vi "SEQU_ChoixGrappe Complete_CN.vi"(3 "indice grappe":u8) -> (1 "Chaîne au format E":string)   [LabVIEW 2022 SP3]
uses:
  TypeDef_Seuil Jauge Pression_CN.ctl
  Voie Analogique_CN.ctl
  Emum Type Jauge de Pression_CN.ctl
  Variables globales/Variable glob Edwards.vi
  Variables globales/Variable glob generale.vi
panel:
  out "Valeur retenue":T1
  out "Seuil Jauge":T3={"Descente en Pression"={"Min Mesure Piezo"=5.0, "Min Mesure Pirani"=0.0002}, "Montée en Pression"={"Max Mesure Pirani"=10.0, "Max Mesure Penning"=0.0004}} {"Montée en Pression"."Max Mesure Penning" format="%.2e"; "Montée en Pression"."Max Mesure Pirani" format="%.2e"; "Descente en Pression"."Min Mesure Pirani" format="%.2e"; "Descente en Pression"."Min Mesure Piezo" format="%.2e"}
  out "Valeurs lues":dbl[](array[numeric])=[1000.0, 1000.0, 4e-10] format="%#_6e"
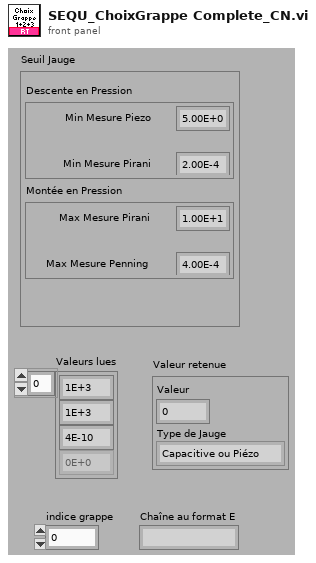
[diagram p1: front panel]
types:
  T1 = typedef "Voie Analogique_CN.ctl" = cluster{"Valeur":dbl, "Type de Jauge":T2}
  T2 = typedef "Emum Type Jauge de Pression_CN.ctl" = enum16{"Capacitive ou Piézo", "Pirani", "Penning"}
  T3 = typedef "TypeDef_Seuil Jauge Pression_CN.ctl" = cluster{"Descente en Pression":cluster{"Min Mesure Piezo":dbl, "Min Mesure Pirani":dbl}, "Montée en Pression":cluster{"Max Mesure Pirani":dbl, "Max Mesure Penning":dbl}}
  T4 = enum16{"Capacitive ou Piézo", "Pirani", "Penning"}
  T5 = enum16{"Capacitive ou Piézo", "Pirani", "Penning", "Bayard Alpert"}
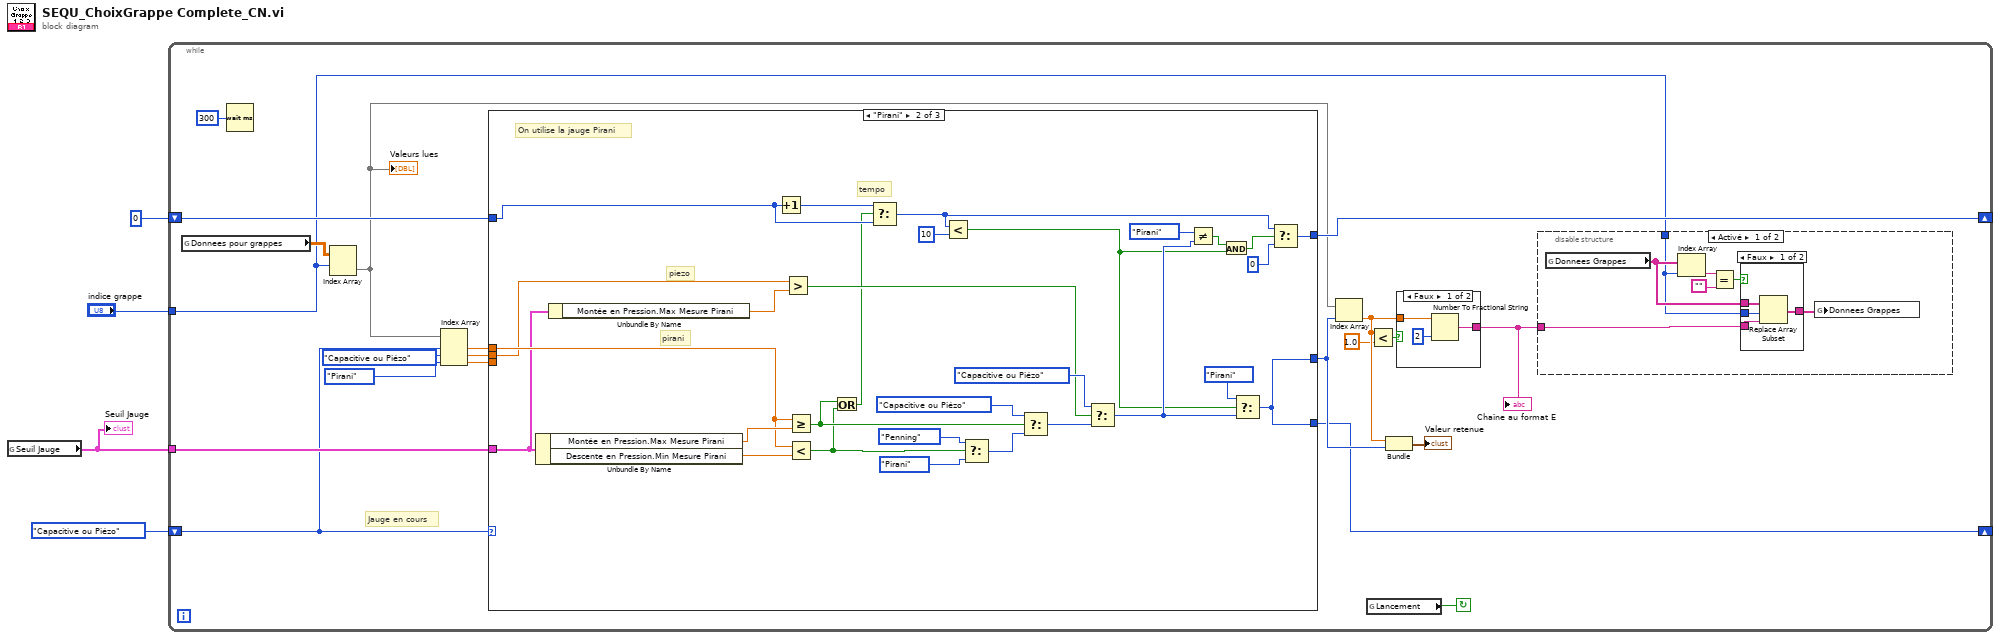
[diagram p0: block diagram]
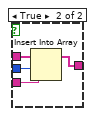
[diagram p2: hidden frame]
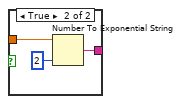
[diagram p4: hidden frame]
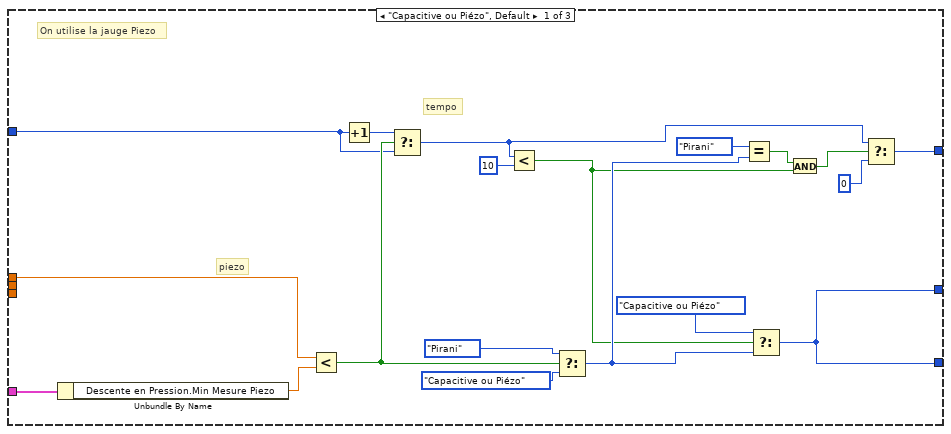
[diagram p5: hidden frame]
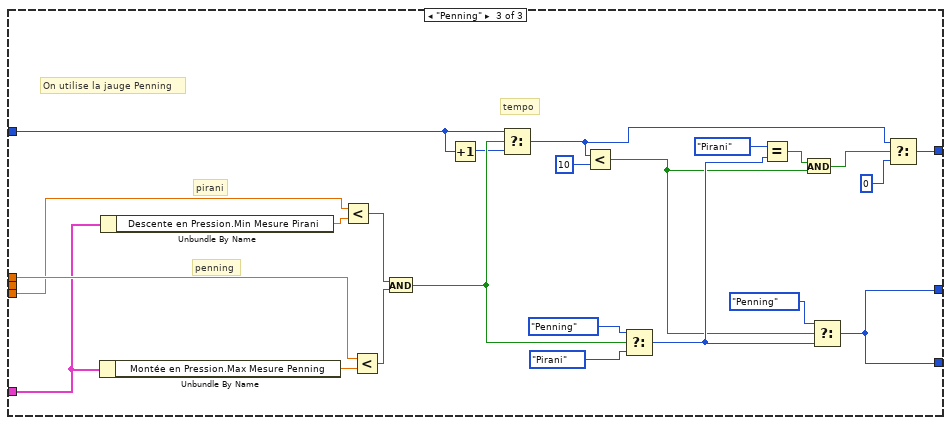
[diagram p6: hidden frame]
diagram:
  n1 = global read "Variable glob Edwards.vi" "Seuil Jauge"() -> (w2:T3)
  "Seuil Jauge" <- w2
  n2 = while {
    tunnel: w2 -> [w25]
    shift-right: [w15] -> _
    shift-left: T4."Capacitive ou Piézo" ("Jauge In") -> [w24]
    shift-right: [w13] -> _
    shift-left: 0 -> [w14]
    tunnel: "indice grappe" -> [w5]
    stop <- w12 continue-if-true
    # "Jauge en cours"
    n3 = global read "Variable glob Edwards.vi" "Donnees pour grappes"() -> (w11:dbl[][])
    n4 = Wait (ms)(milliseconds to wait=u32 300 ("n millisecondes")) -> ()  [unwired: 1 out]
    n5 = Index Array(array=w11, index (row)=w5) -> (element=w10:dbl[])  [unwired: 1 in]
    "Valeurs lues" <- w10
    n6 = Index Array(array=w10, index #1=w24, index #2=T5."Capacitive ou Piézo" ("Jauge In 2"), index #3=T5."Pirani" ("Jauge In 2")) -> (element #1=w23:dbl, element #2=w20:dbl, element #3=w19:dbl)
    n7 = case shown="\"Pirani\"" w24 {
      tunnel: w25 -> [w65 w82 w113]
      tunnel: [w58 w74 w107] -> w16
      tunnel: [w58 w74 w107] -> w15
      tunnel: w23 -> [w61 w88 w114]
      tunnel: w20 -> [_ w86 _]
      tunnel: w19 -> [_ _ w105]
      tunnel: w14 -> [w55 w76 w99]
      tunnel: [w53 w75 w106] -> w13
      frame "Capacitive ou Piézo", Default {
        # "tempo"
        # "piezo"
        # "On utilise la jauge Piezo"
        n8 = Unbundle By Name(w65) -> ("Descente en Pression.Min Mesure Piezo"=w64:dbl)
        n9 = Less?(x=w61, y=w64) -> (x < y?=w57:bool)
        n10 = Increment(x=w55) -> (x+1=w56:i32)
        n11 = Select(t=w56, s=w57, f=w55) -> (s? t:f=w51:i32)
        n12 = Less?(x=w51, y=10) -> (x < y?=w48:bool)
        n13 = Select(t=Emum_Type_Jauge_de_Pression_CN."Pirani" ("Type de Jauge"), s=w57, f=Emum_Type_Jauge_de_Pression_CN."Capacitive ou Piézo" ("Type de Jauge")) -> (s? t:f=w50:T2)
        n14 = Equal?(x=Emum_Type_Jauge_de_Pression_CN."Pirani", y=w50) -> (x = y?=w49:bool)
        n15 = Select(t=Emum_Type_Jauge_de_Pression_CN."Capacitive ou Piézo" ("cas vrai"), s=w48, f=w50) -> (s? t:f=w58:T2)
        n16 = And(x=w49, y=w48) -> (x .and. y?=w47:bool)
        n17 = Select(t=w51, s=w47, f=0 ("cas vrai")) -> (s? t:f=w53:i32)
      }
      frame "Pirani" {
        # "tempo"
        # "piezo"
        # "pirani"
        # "On utilise la jauge Pirani"
        n18 = Unbundle By Name(w82) -> ("Montée en Pression.Max Mesure Pirani"=w94:dbl, "Descente en Pression.Min Mesure Pirani"=w89:dbl)
        n19 = Unbundle By Name(w82) -> ("Montée en Pression.Max Mesure Pirani"=w87:dbl)
        n20 = Increment(x=w76) -> (x+1=w80:i32)
        n21 = Greater?(x=w86, y=w87) -> (0:w73:bool)
        n22 = Greater Or Equal?(x=w88, y=w94) -> (x >= y?=w71:bool)
        n23 = Less?(x=w88, y=w89) -> (x < y?=w70:bool)
        n24 = Or(x=w71, y=w70) -> (x .or. y?=w69:bool)
        n25 = Select(t=w80, s=w69, f=w76) -> (s? t:f=w77:i32)
        n26 = Less?(x=w77, y=10) -> (x < y?=w67:bool)
        n27 = Select(t=Emum_Type_Jauge_de_Pression_CN."Penning" ("Type de Jauge"), s=w70, f=Emum_Type_Jauge_de_Pression_CN."Pirani" ("Type de Jauge")) -> (s? t:f=w92:T2)
        n28 = Select(t=Emum_Type_Jauge_de_Pression_CN."Capacitive ou Piézo" ("Type de Jauge"), s=w71, f=w92) -> (s? t:f=w85:T2)
        n29 = Select(t=Emum_Type_Jauge_de_Pression_CN."Capacitive ou Piézo" ("Type de Jauge"), s=w73, f=w85) -> (s? t:f=w72:T2)
        n30 = Not Equal?(x=Emum_Type_Jauge_de_Pression_CN."Pirani", y=w72) -> (x != y?=w68:bool)
        n31 = And(x=w68, y=w67) -> (x .and. y?=w66:bool)
        n32 = Select(t=Emum_Type_Jauge_de_Pression_CN."Pirani" ("cas vrai"), s=w67, f=w72) -> (s? t:f=w74:T2)
        n33 = Select(t=w77, s=w66, f=0 ("cas vrai")) -> (s? t:f=w75:i32)
      }
      frame "Penning" {
        # "tempo"
        # "pirani"
        # "penning"
        # "On utilise la jauge Penning"
        n34 = Unbundle By Name(w113) -> ("Montée en Pression.Max Mesure Penning"=w115:dbl)
        n35 = Unbundle By Name(w113) -> ("Descente en Pression.Min Mesure Pirani"=w104:dbl)
        n36 = Less?(x=w105, y=w104) -> (x < y?=w103:bool)
        n37 = Less?(x=w114, y=w115) -> (x < y?=w102:bool)
        n38 = And(x=w103, y=w102) -> (x .and. y?=w101:bool)
        n39 = Increment(x=w99) -> (x+1=w100:i32)
        n40 = Select(t=w99, s=w101, f=w100) -> (s? t:f=w108:i32)
        n41 = Less?(x=w108, y=10) -> (x < y?=w96:bool)
        n42 = Select(t=Emum_Type_Jauge_de_Pression_CN."Penning" ("Type de Jauge"), s=w101, f=Emum_Type_Jauge_de_Pression_CN."Pirani" ("Type de Jauge")) -> (s? t:f=w98:T2)
        n43 = Equal?(x=Emum_Type_Jauge_de_Pression_CN."Pirani", y=w98) -> (x = y?=w97:bool)
        n44 = And(x=w97, y=w96) -> (x .and. y?=w95:bool)
        n45 = Select(t=Emum_Type_Jauge_de_Pression_CN."Penning" ("cas vrai"), s=w96, f=w98) -> (s? t:f=w107:T2)
        n46 = Select(t=w108, s=w95, f=0 ("cas vrai")) -> (s? t:f=w106:i32)
      }
    }
    n47 = Index Array(array=w10, index=w16) -> (element=w7:dbl)
    n48 = global read "Variable glob generale.vi" "Lancement"() -> (w12:bool)
    n49 = Less?(x=w7, y=1.0) -> (x < y?=w8:bool)
    n50 = Bundle("Numérique"=w7, "Type de Jauge"=w16) -> (→"Valeur retenue":cluster{"Numérique":dbl, "Type de Jauge":T2})  [unwired: 1 in]
    n51 = case shown="Faux" w8 {
      tunnel: w7 -> [w43 w46]
      tunnel: [w42 w45] -> w9
      frame False {
        n52 = Number To Fractional String(number=w43, precision (6)=i16 2 ("précision (6)")) -> (F-format string=w42:string)  [unwired: 2 in]
      }
      frame True {
        n53 = Number To Exponential String(number=w46, precision (6)=i16 2 ("précision (6)")) -> (E-format string=w45:string)  [unwired: 2 in]
      }
    }
    "Chaîne au format E" <- w9
    n54 = disable-structure shown="Activé" {
      disable-tunnel: w9 -> [w32 _]
      disable-tunnel: w5 -> [w26 _]
      frame Enabled {
        n55 = global read "Variable glob Edwards.vi" "Donnees Grappes"() -> (w30:string[])
        n56 = Index Array(array=w30, index=w26) -> (element=w29:string)
        n57 = Equal?(x=w29, y="") -> (x = y?=w27:bool)
        n58 = case shown="Faux" w27 {
          tunnel: w32 -> [w36 w40]
          tunnel: [w35 w37] -> w31
          tunnel: w30 -> [w34 w39]
          tunnel: w26 -> [w33 w38]
          frame False {
            n59 = Replace Array Subset(array=w34, new element=w36, index=w33) -> (w35:string[])
          }
          frame True {
            n60 = Insert Into Array(array=w39, index=w38, new element=w40) -> (w37:string[])
          }
        }
        n61 = global write "Variable glob Edwards.vi" "Donnees Grappes"(w31) -> ()
      }
      frame Disabled {
      }
    }
  }
